vi "Test Server.vi"() -> ()   [LabVIEW 2013]
uses:
  <vilib>/LabVIEW Open Source Project/MQTT Control Packets/Control Packets/CONNACK/Connect Return Code -- enum.ctl
  <vilib>/LabVIEW Open Source Project/MQTT Control Packets/Control Packets/ControlPacket/QualityOfService -- enum.ctl
  <vilib>/LabVIEW Open Source Project/MQTT Control Packets/Control Packets/CONNECT/ConnectFlags -- cluster.ctl
  source/Server class/Server.lvclass/Server.ctl
  <vilib>/LabVIEW Open Source Project/MQTT Client/Client class/Client.lvclass/Client.ctl
  <vilib>/LabVIEW Open Source Project/MQTT Control Packets/Control Packets/PUBLISH/PUBLISH.lvclass
  source/Server class/Server.lvclass
  <vilib>/LabVIEW Open Source Project/MQTT Connection/MQTT_Base/Base Class/MQTT_Base.lvclass
  <vilib>/LabVIEW Open Source Project/MQTT Client/Client class/Client.lvclass
  <vilib>/LabVIEW Open Source Project/MQTT TCP Connection/MQTT_TCP/Connection/TCPConnection.lvclass
  <vilib>/LabVIEW Open Source Project/MQTT LocalQueue Connection/MQTT_LocalQueue/Connection/LocalQueueConnection.lvclass
  <vilib>/LabVIEW Open Source Project/MQTT Websockets Connection/MQTT_Websockets/Connection/WebsocketsConnection.lvclass
  <vilib>/LabVIEW Open Source Project/MQTT Control Packets/Control Packets/CONNECT/CONNECT.lvclass
  <vilib>/LabVIEW Open Source Project/MQTT Control Packets/Control Packets/CONNACK/CONNACK.lvclass
  <vilib>/LabVIEW Open Source Project/MQTT Control Packets/Control Packets/ControlPacket/ControlPacket.lvclass
panel:
  in  "QoS":T1
  out "Published":bool
  out "Unsuback received":bool
  out "Suback received":bool
  in  "Connection Type":enum16{"TCP", "Local Queue", "WebSockets"}(ring)
  out "error server":errorcluster
  in  "Unsubscribe":bool
  in  "Subscribe":bool
  out "error client sink 2":errorcluster
  out "Random 2":dbl(graph)
  out "received 2":i32
  out "received timer 2":u32
  out "Client Status 2":T2=enum."Server Unavailable"
  out "published timer":u32
  out "received timer":u32
  out "received":i32
  out "published":i32
  out "Random":dbl(graph)
  out "Client Status":T2=enum."Server Unavailable"
  out "error client source":errorcluster
  out "NbConnections":u32
  out "error client sink 1":errorcluster
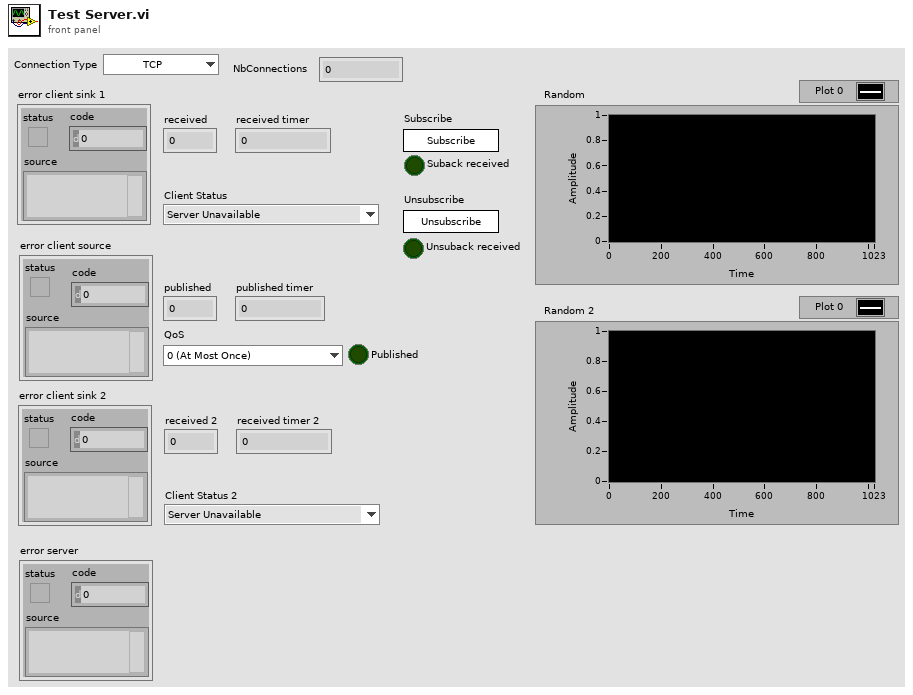
[diagram p1: front panel]
types:
  T1 = typedef "MQTT_Control_Packets.lvlib/ControlPacket.lvclass/QualityOfService -- enum.ctl" = enum16{"0 (At Most Once)", "1 (At Least Once)", "2 (Exactly Once)"}
  T2 = typedef "MQTT_Control_Packets.lvlib/CONNACK.lvclass/Connect Return Code -- enum.ctl" = enum16{"Connection accepted", "Unacceptable protocol version", "Identifier Rejected", "Server Unavailable", "Bad Username or Password", "Not Authorized"}
  T3 = typedef "MQTT_Control_Packets.lvlib/CONNECT.lvclass/ConnectFlags -- cluster.ctl" = cluster{"Reserved":bool, "Clean Session":bool, "Will Flag":bool, "Will QoS 1":bool, "Will QoS 2":bool, "Will Retain":bool, "Password Flag":bool, "User Name Flag":bool}
  T4 = typedef "MQTT Client.lvlib/Client.lvclass/Public Events -- cluster.ctl" = cluster{"Connection Status":refnum<user-event>, "Connected":refnum<user-event>, "Application Message":refnum<user-event>}
  T5 = typedef "MQTT Server.lvlib/Server.lvclass/Public Events -- cluster.ctl" = cluster{"NbConnections":refnum<user-event>}
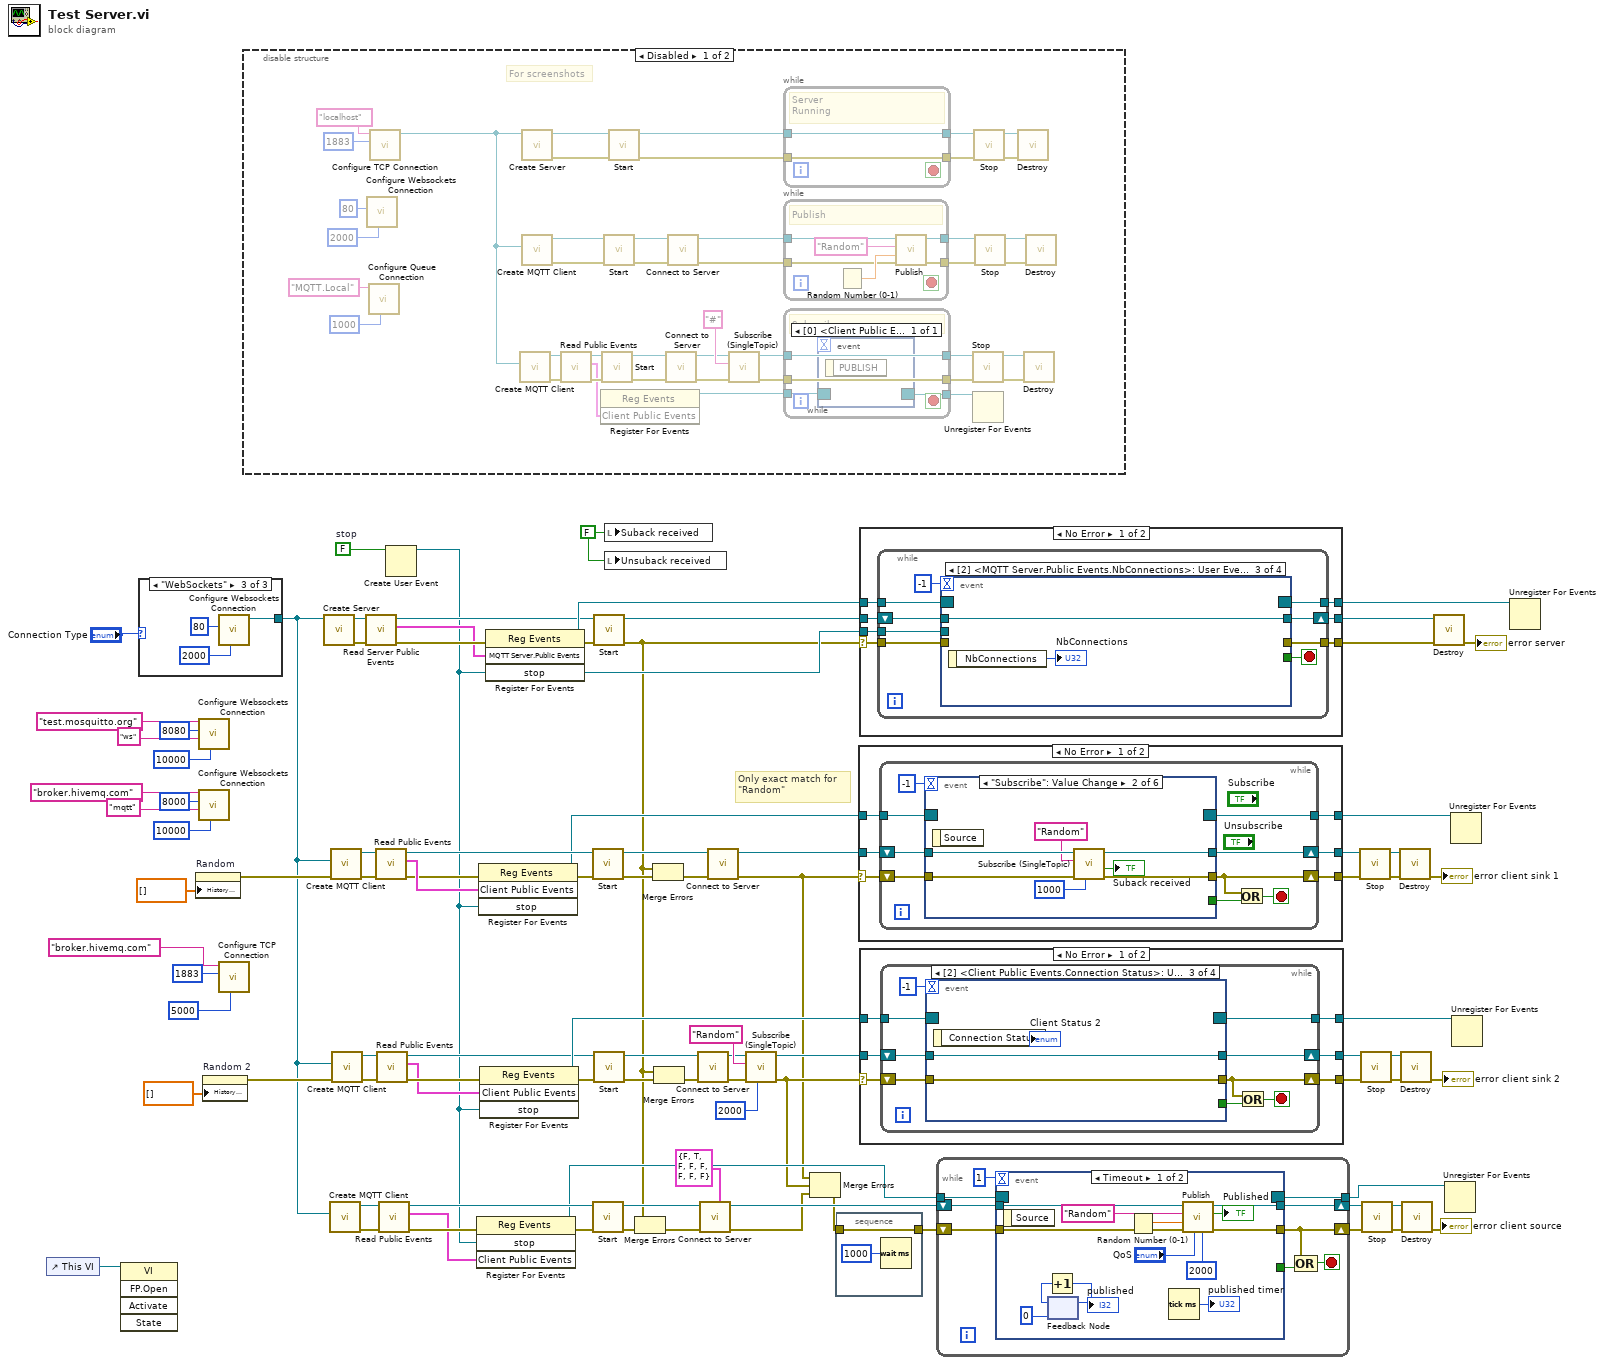
[diagram p0: block diagram]
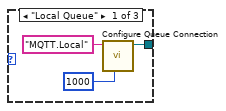
[diagram p2: hidden frame]
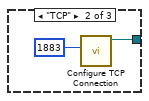
[diagram p3: hidden frame]
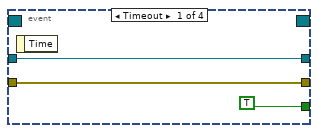
[diagram p5: hidden frame]
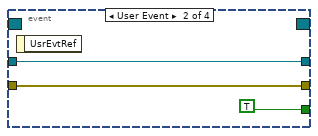
[diagram p6: hidden frame]
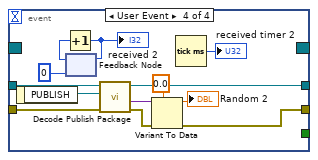
[diagram p7: hidden frame]
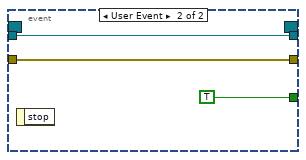
[diagram p9: hidden frame]
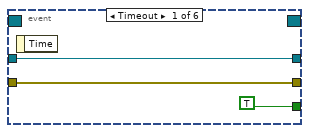
[diagram p10: hidden frame]
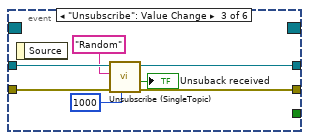
[diagram p11: hidden frame]
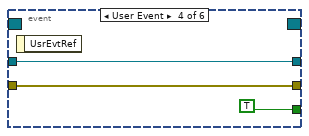
[diagram p12: hidden frame]
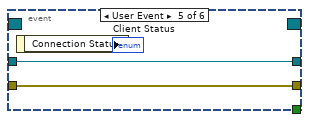
[diagram p13: hidden frame]
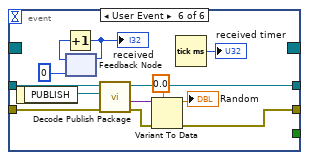
[diagram p14: hidden frame]
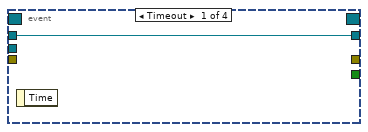
[diagram p16: hidden frame]
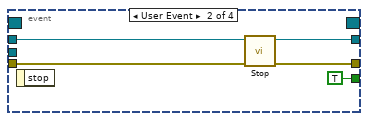
[diagram p17: hidden frame]
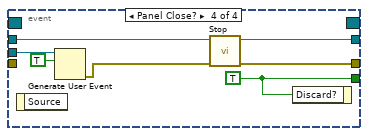
[diagram p18: hidden frame]
diagram:
  w15 = FALSE ("Suback received")
  w53 = FALSE  # stop
  # "Only exact match for\n\"Random\""
  n1 = control-ref of="This VI"() -> (w21:refnum<vi>)
  n2 = invoke class="VI" method="FP.Open"(reference=w21) -> ()  [unwired: 4 in, 5 out]
  n3 = case shown="\"WebSockets\"" "Connection Type" {
    tunnel: [w96 w99 w103] -> w2
    frame "Local Queue" {
      n4 = call <vilib>:"Configure Queue Connection.vi"("timeout (500 ms)"=1000 ("timeout (100ms)"), "Queue Name"="MQTT.Local") -> ("LocalQueueConnection"=w96:refnum<class "LocalQueueConnection.lvclass">)  [unwired: 8 in, 1 out]
    }
    frame "TCP" {
      n5 = call <vilib>:"Configure TCP Connection.vi"("remote port (80)"=u16 1883) -> ("TCPConnection"=w99:refnum<class "TCPConnection.lvclass">)  [unwired: 9 in, 1 out]
    }
    frame "WebSockets" {
      n6 = call <vilib>:"Configure Websockets Connection.vi"("timeout (5000 ms)"=2000 ("timeout (100ms)"), "remote port (80)"=u16 80) -> ("WSConnection"=w103:refnum<class "WebsocketsConnection.lvclass">)  [unwired: 8 in, 1 out]
    }
  }
  n7 = property on="Random" class="WFChart (strict)"("History Data"=dbl[] []) -> (error out=w57:errorcluster)  [unwired: 2 in, 1 out]
  n8 = call <vilib>:"Configure Websockets Connection.vi"("timeout (5000 ms)"=10000 ("timeout (100ms)"), "path"="ws", "remote port (80)"=u16 8080, "address (localhost)"="test.mosquitto.org") -> ()  [unwired: 6 in, 2 out]
  n9 = call <vilib>:"Configure Websockets Connection.vi"("timeout (5000 ms)"=10000 ("timeout (100ms)"), "path"="mqtt", "remote port (80)"=u16 8000, "address (localhost)"="broker.hivemq.com") -> ()  [unwired: 6 in, 2 out]
  n10 = property on="Random 2" class="WFChart (strict)"("History Data"=dbl[] []) -> (error out=w24:errorcluster)  [unwired: 2 in, 1 out]
  n11 = call <vilib>:"Configure TCP Connection.vi"("timeout (5000ms)"=5000 ("timeout (100ms)"), "remote port (80)"=u16 1883, "address (localhost)"="broker.hivemq.com") -> ()  [unwired: 7 in, 2 out]
  n12 = disable-structure shown="Disabled" {
    frame Disabled {
      # "For screenshots"
      n13 = call <vilib>:"Configure Websockets Connection.vi"("timeout (5000 ms)"=2000 ("timeout (100ms)"), "remote port (80)"=u16 80) -> ()  [unwired: 8 in, 2 out]
      n14 = call <vilib>:"Configure Queue Connection.vi"("timeout (500 ms)"=1000 ("timeout (100ms)"), "Queue Name"="MQTT.Local") -> ()  [unwired: 8 in, 2 out]
      n15 = call <vilib>:"Configure TCP Connection.vi"("remote port (80)"=u16 1883, "address (localhost)"="localhost" ("Topic Filter")) -> ("TCPConnection"=w109:refnum<class "TCPConnection.lvclass">)  [unwired: 8 in, 1 out]
      n16 = call <vilib>:"Create MQTT Client.vi"("Connection Configuration"=w109) -> ("error out"=w115:errorcluster, "Client out"=w117:refnum<class "Client.lvclass">)  [unwired: 9 in]
      n17 = call "Create Server.vi"("Connection Configuration"=w109) -> ("error out"=w140:errorcluster, "Server"=w139:refnum<class "Server.lvclass">)  [unwired: 9 in]
      n18 = call <vilib>:"Create MQTT Client.vi"("Connection Configuration"=w109) -> ("error out"=w137:errorcluster, "Client out"=w138:refnum<class "Client.lvclass">)  [unwired: 9 in]
      n19 = call <vilib>:"Read Public Events.vi"("error in (no error)"=w115, "Client in"=w117) -> ("error out"=w114:errorcluster, "Client Public Events"=w113:T4, "Client out"=w116:refnum<class "Client.lvclass">)  [unwired: 7 in]
      n20 = register-events(w113) -> (reference out=w112:refnum<event-registration>)  [unwired: 2 in, 1 out]
      n21 = call <vilib>:"Start.vi"("error in (no error)"=w114, "MQTT_Base in"=w116) -> ("error out"=w132:errorcluster, "MQTT_Base out"=w133:refnum<class "Client.lvclass">)  [unwired: 7 in, 1 out]
      n22 = call <vilib>:"Start.vi"("error in (no error)"=w137, "MQTT_Base in"=w138) -> ("error out"=w144:errorcluster, "MQTT_Base out"=w143:refnum<class "Client.lvclass">)  [unwired: 7 in, 1 out]
      n23 = call <vilib>:"Start.vi"("error in (no error)"=w140, "MQTT_Base in"=w139) -> ("error out"=w124:errorcluster, "MQTT_Base out"=w126:refnum<class "Server.lvclass">)  [unwired: 7 in, 1 out]
      n24 = call <vilib>:"Connect to Server.vi"("error in (no error)"=w132, "Client in"=w133) -> ("error out"=w120:errorcluster, "Client out"=w121:refnum<class "Client.lvclass">)  [unwired: 6 in, 2 out]
      n25 = call <vilib>:"Connect to Server.vi"("error in (no error)"=w144, "Client in"=w143) -> ("error out"=w128:errorcluster, "Client out"=w131:refnum<class "Client.lvclass">)  [unwired: 6 in, 2 out]
      n26 = call <vilib>:"Subscribe (SingleTopic).vi"("error in (no error)"=w120, "Topic Filter"="#", "MQTT_Base in"=w121) -> ("error out"=w118:errorcluster, "MQTT_Base out"=w119:refnum<class "Client.lvclass">)  [unwired: 6 in, 1 out]
      n27 = while {
        tunnel: [w158] -> w127
        tunnel: w126 -> [w158]
        tunnel: w124 -> [w157]
        tunnel: [w157] -> w125
        stop <- _ stop-if-true
        # "Server\nRunning"
      }
      n28 = while {
        tunnel: w131 -> [w154]
        tunnel: [w153] -> w130
        tunnel: [w152] -> w129
        tunnel: w128 -> [w151]
        stop <- _ stop-if-true
        # "Publish"
        n29 = Random Number (0-1)() -> (number: 0 to 1=w156:dbl)
        n30 = call <vilib>:"Publish.vi"("error in (no error)"=w151, "Payload"=w156, "Topic Name (empty: Payload name)"="Random", "Client in"=w154) -> ("error out"=w152:errorcluster, "Client out"=w153:refnum<class "Client.lvclass">)  [unwired: 5 in, 1 out]
      }
      n31 = while {
        tunnel: [w150] -> w122
        tunnel: w119 -> [w150]
        tunnel: w118 -> [w149]
        tunnel: [w149] -> w123
        tunnel: w112 -> [w148]
        tunnel: [w147] -> w111
        stop <- _ stop-if-true
        # "Subscribe"
        n32 = event shown="[0] <Client Public Events.Application Message>: User Event" {
          selector: w148 -> [_]
          dyn-events: [_] -> w147
          timeout: _ -> [_]
          event User Event {
            n33 = event-data() -> ()  [unwired: 1 in, 1 out]
          }
        }
      }
      n34 = call <vilib>:"Stop.vi"("error in (no error)"=w123, "MQTT_Base in"=w122) -> ("error out"=w135:errorcluster, "MQTT_Base out"=w136:refnum<class "Client.lvclass">)  [unwired: 7 in, 1 out]
      n35 = Unregister For Events(event registration refnum=w111) -> ()  [unwired: 1 in, 1 out]
      n36 = call <vilib>:"Stop.vi"("error in (no error)"=w125, "MQTT_Base in"=w127) -> ("error out"=w146:errorcluster, "MQTT_Base out"=w145:refnum<class "Server.lvclass">)  [unwired: 7 in, 1 out]
      n37 = call <vilib>:"Stop.vi"("error in (no error)"=w129, "MQTT_Base in"=w130) -> ("error out"=w142:errorcluster, "MQTT_Base out"=w141:refnum<class "Client.lvclass">)  [unwired: 7 in, 1 out]
      n38 = call <vilib>:"Destroy.vi"("error in (no error)"=w146, "MQTT_Base in"=w145) -> ()  [unwired: 8 in, 2 out]
      n39 = call <vilib>:"Destroy.vi"("error in (no error)"=w135, "MQTT_Base in"=w136) -> ()  [unwired: 8 in, 2 out]
      n40 = call <vilib>:"Destroy.vi"("error in (no error)"=w142, "MQTT_Base in"=w141) -> ()  [unwired: 8 in, 2 out]
    }
    frame Enabled {
    }
  }
  n41 = call "Create Server.vi"("Connection Configuration"=w2) -> ("error out"=w93:errorcluster, "Server"=w94:refnum<class "Server.lvclass">)  [unwired: 9 in]
  n42 = call <vilib>:"Create MQTT Client.vi"("Connection Configuration"=w2) -> ("error out"=w77:errorcluster, "Client out"=w76:refnum<class "Client.lvclass">)  [unwired: 9 in]
  n43 = call <vilib>:"Create MQTT Client.vi"("error in (no error)"=w57, "Connection Configuration"=w2) -> ("error out"=w78:errorcluster, "Client out"=w79:refnum<class "Client.lvclass">)  [unwired: 8 in]
  n44 = call <vilib>:"Create MQTT Client.vi"("error in (no error)"=w24, "Connection Configuration"=w2) -> ("error out"=w29:errorcluster, "Client out"=w28:refnum<class "Client.lvclass">)  [unwired: 8 in]
  n45 = call "Read Server Public Events.vi"("error in (no error)"=w93, "Server in"=w94) -> ("error out"=w92:errorcluster, "MQTT Server.Public Events"=w91:T5, "Server out"=w87:refnum<class "Server.lvclass">)  [unwired: 7 in]
  n46 = call <vilib>:"Read Public Events.vi"("error in (no error)"=w78, "Client in"=w79) -> ("error out"=w62:errorcluster, "Client Public Events"=w63:T4, "Client out"=w75:refnum<class "Client.lvclass">)  [unwired: 7 in]
  n47 = call <vilib>:"Read Public Events.vi"("error in (no error)"=w29, "Client in"=w28) -> ("error out"=w40:errorcluster, "Client Public Events"=w39:T4, "Client out"=w30:refnum<class "Client.lvclass">)  [unwired: 7 in]
  n48 = call <vilib>:"Read Public Events.vi"("error in (no error)"=w77, "Client in"=w76) -> ("error out"=w52:errorcluster, "Client Public Events"=w48:T4, "Client out"=w72:refnum<class "Client.lvclass">)  [unwired: 7 in]
  n49 = Create User Event(user event datatype=w53) -> (user event=w25:refnum<user-event>)  [unwired: 1 in, 1 out]
  n50 = register-events(error in=w52, w25, w48) -> (reference out=w50:refnum<event-registration>, error out=w51:errorcluster)  [unwired: 1 in]
  n51 = register-events(error in=w62, w63, w25) -> (reference out=w60:refnum<event-registration>, error out=w61:errorcluster)  [unwired: 1 in]
  n52 = register-events(error in=w40, w39, w25) -> (reference out=w42:refnum<event-registration>, error out=w41:errorcluster)  [unwired: 1 in]
  n53 = register-events(error in=w92, w91, w25) -> (reference out=w90:refnum<event-registration>, error out=w85:errorcluster)  [unwired: 1 in]
  n54 = call <vilib>:"Start.vi"("error in (no error)"=w61, "MQTT_Base in"=w75) -> ("error out"=w73:errorcluster, "MQTT_Base out"=w74:refnum<class "Client.lvclass">)  [unwired: 7 in, 1 out]
  n55 = call <vilib>:"Start.vi"("error in (no error)"=w51, "MQTT_Base in"=w72) -> ("error out"=w70:errorcluster, "MQTT_Base out"=w71:refnum<class "Client.lvclass">)  [unwired: 7 in, 1 out]
  n56 = call <vilib>:"Start.vi"("error in (no error)"=w85, "MQTT_Base in"=w87) -> ("error out"=w23:errorcluster, "MQTT_Base out"=w86:refnum<class "Server.lvclass">)  [unwired: 7 in, 1 out]
  n57 = call <vilib>:"Start.vi"("error in (no error)"=w41, "MQTT_Base in"=w30) -> ("error out"=w32:errorcluster, "MQTT_Base out"=w31:refnum<class "Client.lvclass">)  [unwired: 7 in, 1 out]
  n58 = local write "Suback received"(w15) -> ()
  n59 = local write "Unsuback received"(w15) -> ()
  n60 = Merge Errors(w23, w70) -> (w80:errorcluster)
  n61 = Merge Errors(w23, w73) -> (w81:errorcluster)
  n62 = Merge Errors(w23, w32) -> (w27:errorcluster)
  n63 = call <vilib>:"Connect to Server.vi"("error in (no error)"=w27, "Client in"=w31) -> ("error out"=w36:errorcluster, "Client out"=w35:refnum<class "Client.lvclass">)  [unwired: 6 in, 2 out]
  n64 = call <vilib>:"Connect to Server.vi"("Connect Flags"=T3 {"Reserved"=FALSE, "Clean Session"=TRUE, "Will Flag"=FALSE, "Will QoS 1"=FALSE, "Will QoS 2"=FALSE, "Will Retain"=FALSE, "Password Flag"=FALSE, "User Name Flag"=FALSE}, "error in (no error)"=w80, "Client in"=w71) -> ("error out"=w47:errorcluster, "Client out"=w88:refnum<class "Client.lvclass">)  [unwired: 5 in, 2 out]
  n65 = call <vilib>:"Connect to Server.vi"("error in (no error)"=w81, "Client in"=w74) -> ("error out"=w18:errorcluster, "Client out"=w19:refnum<class "Client.lvclass">)  [unwired: 6 in, 2 out]
  n66 = call <vilib>:"Subscribe (SingleTopic).vi"("timeout (100ms)"=2000, "error in (no error)"=w36, "Topic Filter"="Random", "MQTT_Base in"=w35) -> ("error out"=w22:errorcluster, "MQTT_Base out"=w44:refnum<class "Client.lvclass">)  [unwired: 5 in, 1 out]
  n67 = Merge Errors(w18, w22, w47) -> (w55:errorcluster)
  n68 = stacked-sequence {
    tunnel: [w159] -> w54
    tunnel: w55 -> [w159]
    frame #0 {
      n69 = Wait (ms)(milliseconds to wait=u32 1000) -> ()  [unwired: 1 out]
    }
  }
  n70 = case shown="No Error" w18 {
    selector: w18 -> [w161 w212]
    tunnel: w60 -> [w166 w214]
    tunnel: [w165 w214] -> w59
    tunnel: w19 -> [w164 w213]
    tunnel: [w163 w213] -> w58
    tunnel: [w162 w212] -> w56
    frame No Error {
      n71 = while {
        tunnel: w166 -> [w175]
        tunnel: [w174] -> w165
        shift-right: [w172] -> w163
        shift-left: w164 -> [w173]
        shift-right: [w169] -> w162
        shift-left: w161 -> [w171]
        stop <- w170 stop-if-true
        n72 = event shown="[1] \"Subscribe\": Value Change" {
          selector: w175 -> [_ _ _ _ _ _]
          dyn-events: [_ _ _ _ _ _] -> w174
          timeout: -1 -> [_ _ _ _ _ _]
          tunnel: w173 -> [w177 w185 w192 w194 w197 w210]
          tunnel: [w177 w182 w191 w194 w197 w206] -> w172
          tunnel: [w176 w181 w188 w193 w196 w199] -> w169
          tunnel: w171 -> [w176 w184 w189 w193 w196 w205]
          tunnel: [TRUE _ _ TRUE _ _] -> w168
          event Timeout {
            n73 = event-data() -> ()  [unwired: 1 in, 1 out]
          }
          event "Subscribe": Value Change {
            n74 = event-data() -> ()  [unwired: 1 in, 1 out]
            n75 = call <vilib>:"Subscribe (SingleTopic).vi"("timeout (100ms)"=1000, "error in (no error)"=w184, "Topic Filter"="Random", "MQTT_Base in"=w185) -> ("error out"=w181:errorcluster, "Ack"=→"Suback received":bool, "MQTT_Base out"=w182:refnum<class "Client.lvclass">)  [unwired: 5 in]
          }
          event "Unsubscribe": Value Change {
            n76 = event-data() -> ()  [unwired: 1 in, 1 out]
            n77 = call <vilib>:"Unsubscribe (SingleTopic).vi"("timeout (100ms)"=1000, "error in (no error)"=w189, "Topic Filter"="Random", "MQTT_Base in"=w192) -> ("error out"=w188:errorcluster, "Ack"=→"Unsuback received":bool, "MQTT_Base out"=w191:refnum<class "Client.lvclass">)  [unwired: 5 in]
          }
          event User Event {
            n78 = event-data() -> ()  [unwired: 1 in, 1 out]
          }
          event User Event {
            n79 = event-data() -> ("Connection Status"=→"Client Status":T2)  [unwired: 1 in]
          }
          event User Event {
            n80 = event-data() -> ("PUBLISH"=w211:refnum<class "PUBLISH.lvclass">)  [unwired: 1 in]
            n81 = feedback #1(0 ("received")) -> (w203:i32)
            n82 = Increment(x=w203) -> (x+1=w202:i32)
            "received" <- w202
            n83 = feedback-in #1(w202) -> ()
            n84 = call <vilib>:"Decode Publish Package.vi"("error in (no error)"=w205, "PUBLISH"=w211, "MQTT_Base in"=w210) -> ("error out"=w200:errorcluster, "Payload"=w209:variant, "MQTT_Base out"=w206:refnum<class "Client.lvclass">)  [unwired: 5 in, 1 out]
            n85 = Variant To Data(error in=w200, type=0.0, Variant=w209) -> (data=→"Random":dbl, error out=w199:errorcluster)
            n86 = Tick Count (ms)() -> (millisecond timer value=→"received timer":u32)
          }
        }
        n87 = Or(x=w169, y=w168) -> (x .or. y?=w170:bool)
      }
    }
    frame Error {
    }
  }
  n88 = case shown="No Error" w23 {
    selector: w23 -> [w215 w246]
    tunnel: w86 -> [w221 w248]
    tunnel: [w220 w248] -> w95
    tunnel: w90 -> [w219 w247]
    tunnel: [w218 w247] -> w89
    tunnel: [w217 w246] -> w84
    tunnel: w25 -> [w216 _]
    frame No Error {
      n89 = while {
        shift-right: [w227] -> w220
        shift-left: w221 -> [w229]
        tunnel: w219 -> [w226]
        tunnel: [w225] -> w218
        tunnel: [w224] -> w217
        tunnel: w216 -> [w223]
        tunnel: w215 -> [w222]
        stop <- w228 stop-if-true
        n90 = event shown="[2] <MQTT Server.Public Events.NbConnections>: User Event" {
          selector: w226 -> [_ _ _ _]
          dyn-events: [_ _ _ _] -> w225
          timeout: -1 -> [_ _ _ _]
          tunnel: w229 -> [w231 w236 w238 w245]
          tunnel: [_ TRUE ("Discard?") _ w244] -> w228
          tunnel: [w231 w235 w238 w243] -> w227
          tunnel: [_ w234 _ w242] -> w224
          tunnel: w223 -> [_ _ _ w241]
          tunnel: w222 -> [_ w232 _ _]
          event Timeout {
            n91 = event-data() -> ()  [unwired: 1 in, 1 out]
          }
          event User Event {
            n92 = event-data() -> ()  [unwired: 1 in, 1 out]
            n93 = call <vilib>:"Stop.vi"("error in (no error)"=w232, "MQTT_Base in"=w236) -> ("error out"=w234:errorcluster, "MQTT_Base out"=w235:refnum<class "Server.lvclass">)  [unwired: 7 in, 1 out]
          }
          event User Event {
            n94 = event-data() -> ("NbConnections"=→"NbConnections":u32)  [unwired: 1 in]
          }
          event Panel Close? {
            w244 = TRUE ("Discard?")
            n95 = event-data() -> ()  [unwired: 1 in, 1 out]
            n96 = Generate User Event(user event=w241, event data cluster=TRUE ("event data")) -> (error out=w239:errorcluster)  [unwired: 2 in, 1 out]
            n97 = call <vilib>:"Stop.vi"("error in (no error)"=w239, "MQTT_Base in"=w245) -> ("error out"=w242:errorcluster, "MQTT_Base out"=w243:refnum<class "Server.lvclass">)  [unwired: 7 in, 1 out]
            n98 = event-data("Discard?"=w244) -> ()  [unwired: 1 in, 1 out]
          }
        }
      }
    }
    frame Error {
    }
  }
  n99 = case shown="No Error" w22 {
    selector: w22 -> [w249 w286]
    tunnel: w42 -> [w254 w288]
    tunnel: [w253 w288] -> w43
    tunnel: w44 -> [w252 w287]
    tunnel: [w251 w287] -> w45
    tunnel: [w250 w286] -> w46
    frame No Error {
      n100 = while {
        tunnel: w254 -> [w263]
        tunnel: [w262] -> w253
        shift-right: [w260] -> w251
        shift-left: w252 -> [w261]
        shift-right: [w257] -> w250
        shift-left: w249 -> [w259]
        stop <- w258 stop-if-true
        n101 = event shown="[2] <Client Public Events.Connection Status>: User Event" {
          selector: w263 -> [_ _ _ _]
          dyn-events: [_ _ _ _] -> w262
          timeout: -1 -> [_ _ _ _]
          tunnel: w261 -> [w265 w268 w271 w284]
          tunnel: [w265 w268 w271 w280] -> w260
          tunnel: [w264 w267 w270 w273] -> w257
          tunnel: w259 -> [w264 w267 w270 w279]
          tunnel: [TRUE TRUE _ _] -> w256
          event Timeout {
            n102 = event-data() -> ()  [unwired: 1 in, 1 out]
          }
          event User Event {
            n103 = event-data() -> ()  [unwired: 1 in, 1 out]
          }
          event User Event {
            n104 = event-data() -> ("Connection Status"=→"Client Status 2":T2)  [unwired: 1 in]
          }
          event User Event {
            n105 = event-data() -> ("PUBLISH"=w285:refnum<class "PUBLISH.lvclass">)  [unwired: 1 in]
            n106 = feedback #2(0 ("received")) -> (w277:i32)
            n107 = Increment(x=w277) -> (x+1=w276:i32)
            "received 2" <- w276
            n108 = feedback-in #2(w276) -> ()
            n109 = call <vilib>:"Decode Publish Package.vi"("error in (no error)"=w279, "PUBLISH"=w285, "MQTT_Base in"=w284) -> ("error out"=w274:errorcluster, "Payload"=w283:variant, "MQTT_Base out"=w280:refnum<class "Client.lvclass">)  [unwired: 5 in, 1 out]
            n110 = Variant To Data(error in=w274, type=0.0, Variant=w283) -> (data=→"Random 2":dbl, error out=w273:errorcluster)
            n111 = Tick Count (ms)() -> (millisecond timer value=→"received timer 2":u32)
          }
        }
        n112 = Or(x=w257, y=w256) -> (x .or. y?=w258:bool)
      }
    }
    frame Error {
    }
  }
  n113 = while {
    shift-right: [w296] -> w69
    shift-left: w88 -> [w297]
    shift-right: [w289] -> w49
    shift-left: w54 -> [w295]
    tunnel: w50 -> [w293]
    tunnel: [w291] -> w20
    stop <- w294 stop-if-true
    n114 = event shown="[0] Timeout" {
      selector: w293 -> [_ _]
      dyn-events: [_ _] -> w291
      timeout: 1 -> [_ _]
      tunnel: w297 -> [w306 w311]
      tunnel: [w305 w311] -> w296
      tunnel: w295 -> [w304 w312]
      tunnel: [w303 w312] -> w289
      tunnel: [_ TRUE] -> w292
      event Timeout {
        n115 = event-data() -> ()  [unwired: 1 in, 1 out]
        n116 = feedback #3(0 ("received")) -> (w309:i32)
        n117 = Increment(x=w309) -> (x+1=w307:i32)
        "published" <- w307
        n118 = feedback-in #3(w307) -> ()
        n119 = Random Number (0-1)() -> (number: 0 to 1=w301:dbl)
        n120 = Tick Count (ms)() -> (millisecond timer value=→"published timer":u32)
        n121 = call <vilib>:"Publish.vi"("timeout (1000ms)"=2000, "QoS"="QoS", "error in (no error)"=w304, "Payload"=w301, "Topic Name (empty: Payload name)"="Random", "Client in"=w306) -> ("error out"=w303:errorcluster, "Published"=→"Published":bool, "Client out"=w305:refnum<class "Client.lvclass">)  [unwired: 3 in]
      }
      event User Event {
        n122 = event-data() -> ()  [unwired: 1 in, 1 out]
      }
    }
    n123 = Compound Arithmetic op=OR(w289, w292) -> (w294:bool)
  }
  n124 = call <vilib>:"Stop.vi"("error in (no error)"=w56, "MQTT_Base in"=w58) -> ("error out"=w66:errorcluster, "MQTT_Base out"=w65:refnum<class "Client.lvclass">)  [unwired: 7 in, 1 out]
  n125 = call <vilib>:"Stop.vi"("error in (no error)"=w46, "MQTT_Base in"=w45) -> ("error out"=w33:errorcluster, "MQTT_Base out"=w34:refnum<class "Client.lvclass">)  [unwired: 7 in, 1 out]
  n126 = call <vilib>:"Stop.vi"("error in (no error)"=w49, "MQTT_Base in"=w69) -> ("error out"=w67:errorcluster, "MQTT_Base out"=w68:refnum<class "Client.lvclass">)  [unwired: 7 in, 1 out]
  n127 = call <vilib>:"Destroy.vi"("error in (no error)"=w66, "MQTT_Base in"=w65) -> ("error out"=→"error client sink 1":errorcluster)  [unwired: 8 in, 1 out]
  n128 = call <vilib>:"Destroy.vi"("error in (no error)"=w33, "MQTT_Base in"=w34) -> ("error out"=→"error client sink 2":errorcluster)  [unwired: 8 in, 1 out]
  n129 = call <vilib>:"Destroy.vi"("error in (no error)"=w67, "MQTT_Base in"=w68) -> ("error out"=→"error client source":errorcluster)  [unwired: 8 in, 1 out]
  n130 = call <vilib>:"Destroy.vi"("error in (no error)"=w84, "MQTT_Base in"=w95) -> ("error out"=→"error server":errorcluster)  [unwired: 8 in, 1 out]
  n131 = Unregister For Events(event registration refnum=w20) -> ()  [unwired: 1 in, 1 out]
  n132 = Unregister For Events(event registration refnum=w59) -> ()  [unwired: 1 in, 1 out]
  n133 = Unregister For Events(event registration refnum=w43) -> ()  [unwired: 1 in, 1 out]
  n134 = Unregister For Events(event registration refnum=w89) -> ()  [unwired: 1 in, 1 out]
